vi "RDC-saltwater-generate_parameter.vi"() -> (0 "defalut":T1={"temp Cx10"=250, "eps s"=76.16, "eps infi"=5.2, "tau"=7.867e-12, "alpha"=0.0102, "sigma"=1.545, "eps s diff"=0.2, "eps infi diff"=0.1, "tau diff"=5e-14, "alpha diff"=0.001, "sigma diff"=0.01}, 3 "map":map{i32, T1}(c390))   [LabVIEW 2020, in "RDC-Reflection_Data_Computation.lvlib"]
doc: "Builds a map of salt water model parameters per temperature (eps s, eps infi, tau, alpha, sigma) by interpolating the table from RDC-saltwater-read_parameter. Also returns a default parameter set."
uses:
  RDC-Reflection_Data_Computation.lvlib
  <vilib>/gmath/NI_Gmath.lvlib
  RDC-saltwater-param.ctl
panel:
  out "temp":dbl[](array[numeric])
  out "temp used":dbl[][](array[numeric])
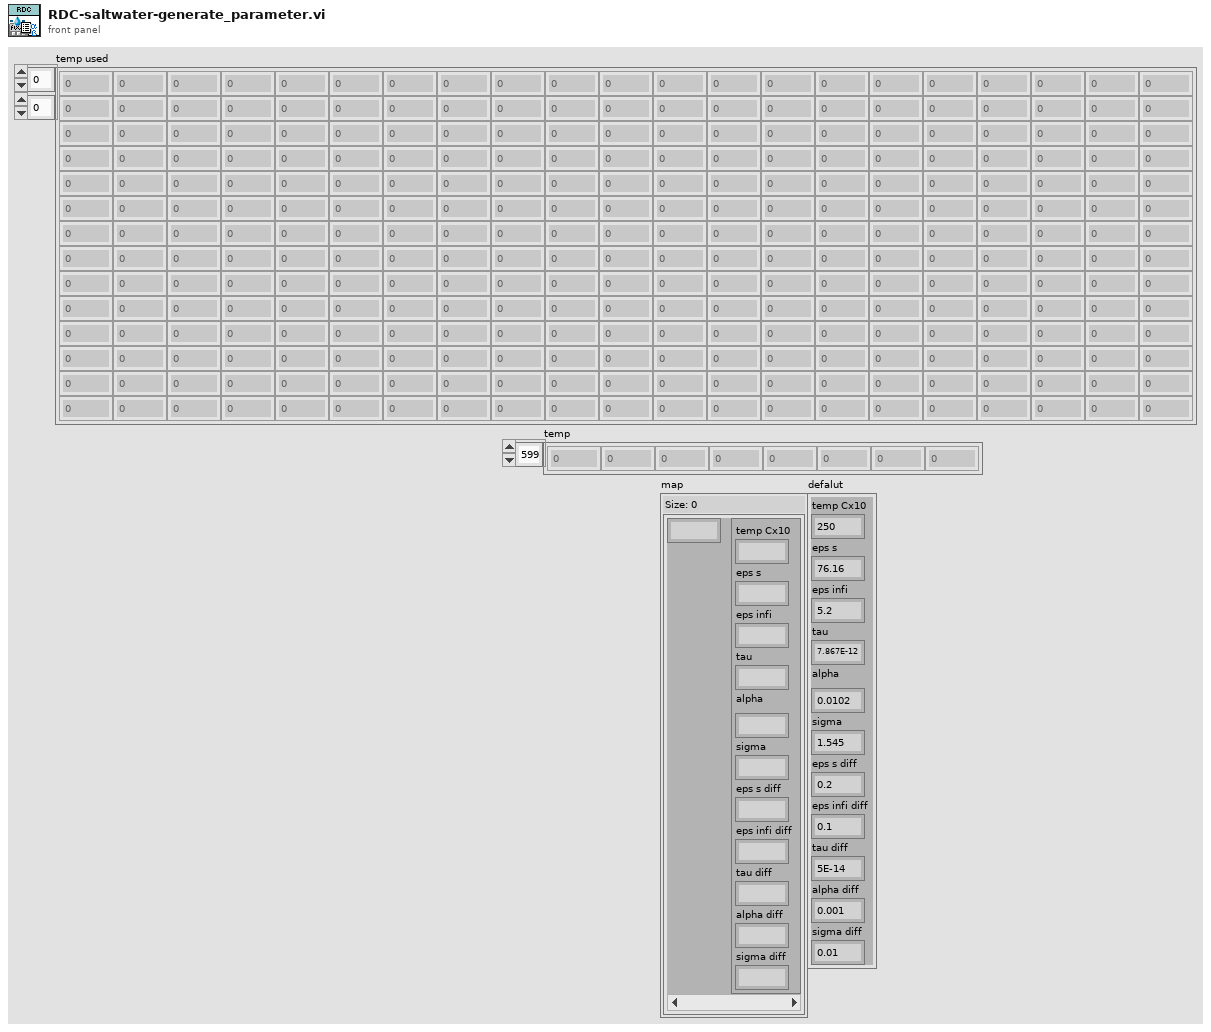
[diagram p1: front panel]
types:
  T1 = typedef "RDC-Reflection_Data_Computation.lvlib/RDC-saltwater-param.ctl" = cluster{"temp Cx10":u16, "eps s":dbl, "eps infi":dbl, "tau":dbl, "alpha":dbl, "sigma":dbl, "eps s diff":dbl, "eps infi diff":dbl, "tau diff":dbl, "alpha diff":dbl, "sigma diff":dbl}
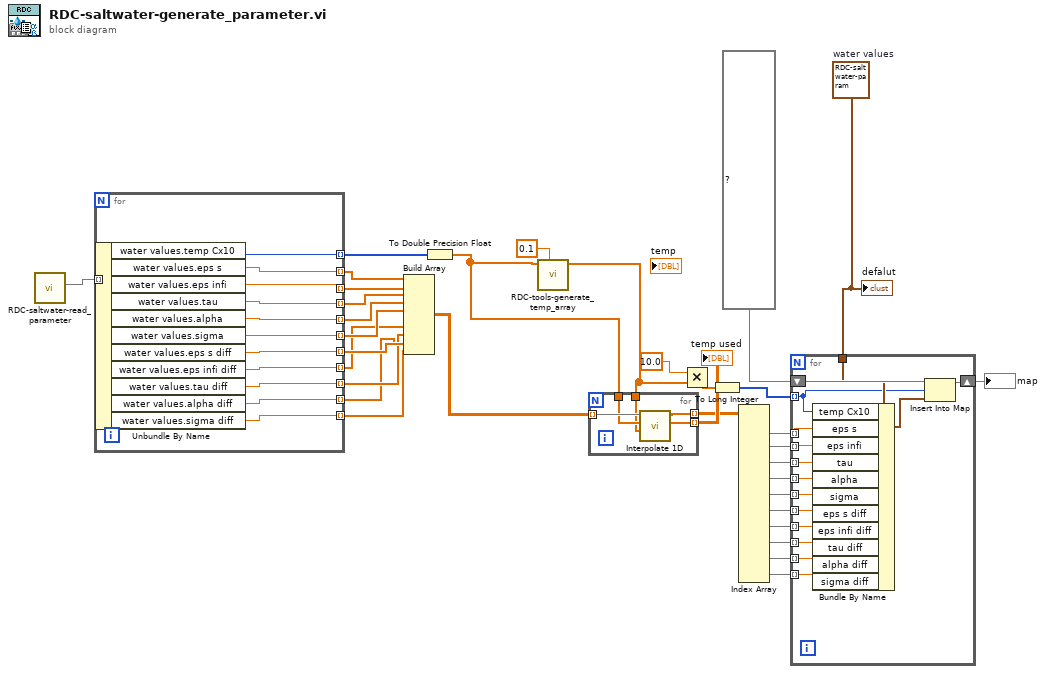
[diagram p0: block diagram]
diagram:
  w2 = T1 {"temp Cx10"=250, "eps s"=76.16, "eps infi"=5.2, "tau"=7.867e-12, "alpha"=0.0102, "sigma"=1.545, "eps s diff"=0.2, "eps infi diff"=0.1, "tau diff"=5e-14, "alpha diff"=0.001, "sigma diff"=0.01}  # water values
  n1 = call "RDC-saltwater-read_parameter.vi"() -> ("map"=w16:map{u16, T1})  [unwired: 10 in, 1 out]
  n2 = for {
    tunnel: w16 -> [w46] mode=indexing
    tunnel: [w44] -> w33 mode=indexing
    tunnel: [w43] -> w32 mode=indexing
    tunnel: [w42] -> w31 mode=indexing
    tunnel: [w45] -> w6 mode=indexing
    tunnel: [w41] -> w29 mode=indexing
    tunnel: [w40] -> w28 mode=indexing
    tunnel: [w39] -> w27 mode=indexing
    tunnel: [w38] -> w15 mode=indexing
    tunnel: [w37] -> w14 mode=indexing
    tunnel: [w36] -> w13 mode=indexing
    tunnel: [w35] -> w12 mode=indexing
    n3 = Unbundle By Name(w46) -> ("water values.temp Cx10"=w45:u16, "water values.eps s"=w44:dbl, "water values.eps infi"=w43:dbl, "water values.tau"=w42:dbl, "water values.alpha"=w41:dbl, "water values.sigma"=w40:dbl, "water values.eps s diff"=w39:dbl, "water values.eps infi diff"=w38:dbl, "water values.tau diff"=w37:dbl, "water values.alpha diff"=w36:dbl, "water values.sigma diff"=w35:dbl)
  }
  n4 = Build Array(w33, w32, w31, w29, w28, w27, w15, w14, w13, w12) -> (w34:dbl[][])
  n5 = To Double Precision Float(number=w6) -> (double precision float=w4:dbl[])
  n6 = call "RDC-tools-generate_temp_array.vi"("Increment"=0.1 ("y"), "temp Cx10"=w4) -> ("temp C"=w3:dbl[])  [unwired: 9 in]
  n7 = for {
    tunnel: w34 -> [w51] mode=indexing
    tunnel: [w50] -> w26 mode=indexing
    tunnel: w4 -> [w49]
    tunnel: [w48] -> w30 mode=indexing
    tunnel: w3 -> [w47]
    n8 = call <vilib>:"Interpolate 1D.vi"("xi"=w47, "X"=w49, "Y"=w51) -> ("xi used"=w48:dbl[], "yi"=w50:dbl[])  [unwired: 6 in, 1 out]
  }
  "temp used" <- w30
  n9 = Multiply(x=10.0 ("temp C"), y=w3) -> (x*y=w18:dbl[])
  n10 = To Long Integer(number=w18) -> (32bit integer=w25:i32[])
  n11 = Index Array(array=w26) -> (element #1=w24:dbl[], element #2=w23:dbl[], element #3=w22:dbl[], element #4=w21:dbl[], element #5=w20:dbl[], element #6=w19:dbl[], element #7=w10:dbl[], element #8=w9:dbl[], element #9=w8:dbl[], element #10=w7:dbl[])  [unwired: 20 in]
  n12 = for {
    tunnel: w25 -> [w63] mode=indexing
    tunnel: w24 -> [w60] mode=indexing
    tunnel: w23 -> [w61] mode=indexing
    tunnel: w22 -> [w62] mode=indexing
    tunnel: w21 -> [w58] mode=indexing
    tunnel: w20 -> [w57] mode=indexing
    tunnel: w19 -> [w56] mode=indexing
    shift-right: [w59] -> w11
    shift-left: map{i32, T1} {} ("map") -> [w66]
    tunnel: w2 -> [w65]
    tunnel: w10 -> [w55] mode=indexing
    tunnel: w9 -> [w54] mode=indexing
    tunnel: w8 -> [w53] mode=indexing
    tunnel: w7 -> [w52] mode=indexing
    n13 = Bundle By Name(cluster=w65, "temp Cx10"=w63, "eps s"=w60, "eps infi"=w61, "tau"=w62, "alpha"=w58, "sigma"=w57, "eps s diff"=w56, "eps infi diff"=w55, "tau diff"=w54, "alpha diff"=w53, "sigma diff"=w52) -> (w64:T1)
    n14 = Insert Into Map(map in=w66, key=w63, value=w64) -> (map out=w59:map{i32, T1})  [unwired: 2 out]
  }
  "map" <- w11
  "defalut" <- w2
